vi "Write Raw.vi"(8 "error in (no error)":errorcluster, 10 "Path":path, 11 "ImageHandler:Varex-ImageHandler in":refnum<class "Varex-ImageHandler.lvclass">) -> (0 "error out":errorcluster, 3 "ImageHandler:Varex-ImageHandler out":refnum<class "Varex-ImageHandler.lvclass">)   [LabVIEW 2022 SP3, in "ImageHandler.lvlib" / "Varex-ImageHandler.lvclass"]
uses:
  Varex-ImageHandler.lvclass
  Varex-ImageHandler.lvclass/Varex-ImageHandler.ctl
  <vilib>/vision/Image Controls.llb/IMAQ Image.ctl
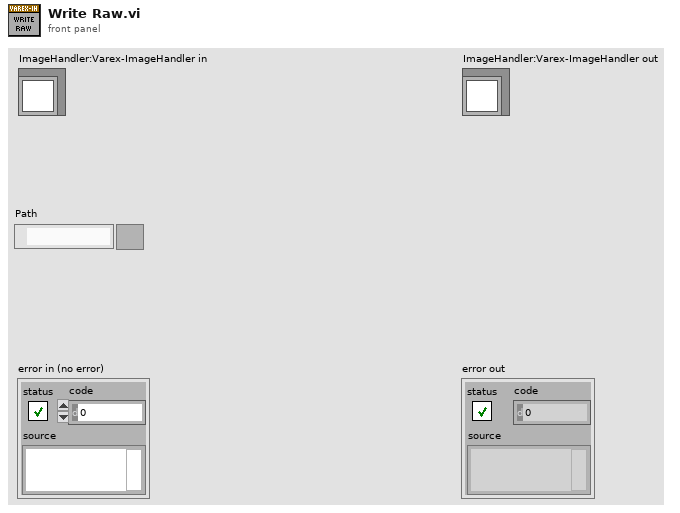
[diagram p1: front panel]
types:
  T1 = enum16{"open", "replace", "create", "open or create", "replace or create", "replace or create with confirmation"}
  T2 = typedef "IMAQ Image.ctl" = refnum<image>
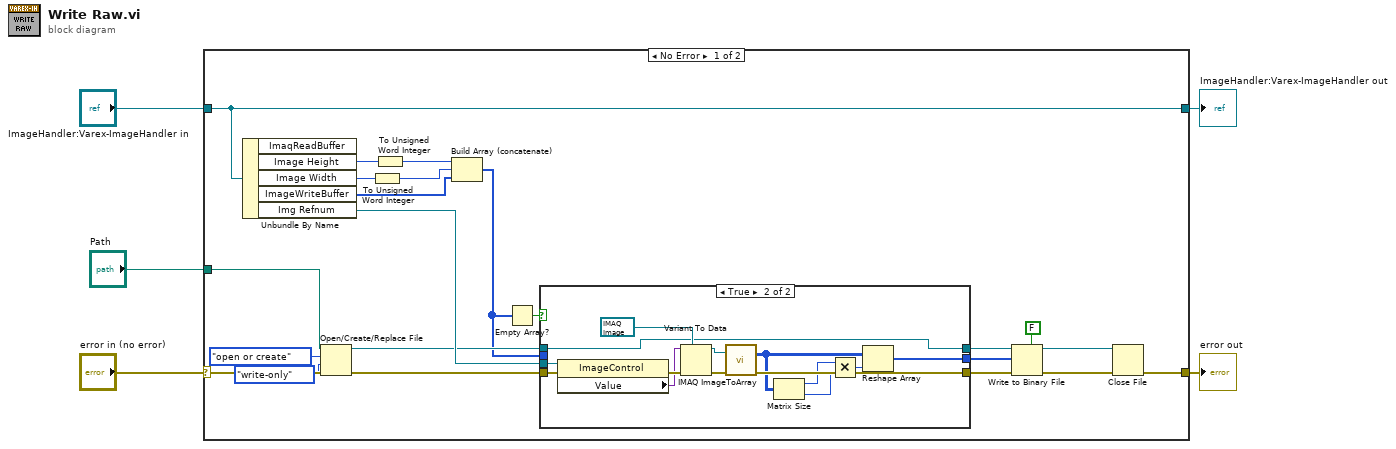
[diagram p0: block diagram]
diagram:
  n1 = case shown="No Error" "error in (no error)" {
    selector: "error in (no error)" -> [w27 w46]
    tunnel: [w24 w46] -> w4
    tunnel: [w26 w45] -> w2
    tunnel: "ImageHandler:Varex-ImageHandler in" -> [w26 w45]
    tunnel: "Path" -> [w23 _]
    frame No Error {
      n2 = Unbundle By Name(w26) -> ("Image Height"=w21:i32, "Image Width"=w20:i32, "ImageWriteBuffer"=w19:u16[], "Img Refnum"=w10:refnum<vi>)  [unwired: 1 out]
      n3 = Open/Create/Replace File(file path (use dialog)=w23, error in=w27, operation (0:open)=T1."open or create", access (0:read/write)=enum16{"read/write", "read-only", "write-only"}."write-only") -> (refnum out=w7:refnum<file>, error out=w12:errorcluster)  [unwired: 2 in, 1 out]
      n4 = To Unsigned Word Integer(number=w20) -> (unsigned 16bit integer=w17:u16)
      n5 = To Unsigned Word Integer(number=w21) -> (unsigned 16bit integer=w18:u16)
      n6 = Build Array (concatenate)(w18, w17, w19) -> (w6:u16[])
      n7 = Empty Array?(array=w6) -> (empty?=w15:bool)
      n8 = case shown="True" w15 {
        tunnel: [w30 w38] -> w11
        tunnel: w12 -> [w30 w44]
        tunnel: w10 -> [_ w42]
        tunnel: [w28 w36] -> w9
        tunnel: [w29 w34] -> w8
        tunnel: w7 -> [w29 w34]
        tunnel: w6 -> [w28 _]
        frame False {
        }
        frame True {
          n9 = property class="ImageControl"(reference=w42, error in=w44) -> (error out=w43:errorcluster, "Value"=w40:variant)  [unwired: 1 out]
          n10 = Variant To Data(error in=w43, type=T2 refnum ("ImaqReadBuffer"), Variant=w40) -> (data=w37:T2, error out=w41:errorcluster)
          n11 = call "IMAQ ImageToArray"("error in (no error)"=w41, "Image"=w37) -> ("Image Pixels (U16)"=w35:u16[][], "error out"=w38:errorcluster)  [unwired: 2 in, 3 out]
          n12 = Matrix Size(0:w35) -> (1:w31:i32, 2:w32:i32)
          n13 = Multiply(x=w31, y=w32) -> (x*y=w33:i32)
          n14 = Reshape Array(w35, w33) -> (w36:u16[])
        }
      }
      n15 = Write to Binary File(file (use dialog)=w8, data=w9, error in=w11, 5:FALSE ("prepend array or string size? (T)")) -> (refnum out=w22:refnum<file>, error out=w25:errorcluster)  [unwired: 2 in, 1 out]
      n16 = Close File(refnum=w22, error in=w25) -> (error out=w24:errorcluster)  [unwired: 1 out]
    }
    frame Error {
    }
  }
  "error out" <- w4
  "ImageHandler:Varex-ImageHandler out" <- w2
